vi "Caller.vi"(0 "x":dbl) -> (1 "y":dbl)   [LabVIEW 2026]
doc: "Probe fixture: calls Callee.vi once."
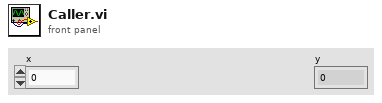
[diagram p1: front panel]
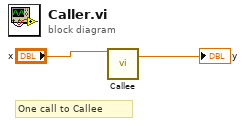
[diagram p0: block diagram]
diagram:
  # "One call to Callee"
  n1 = call "Callee.vi"("x"="x") -> ("y"=→"y":dbl)  [unwired: 14 in]
